vi "Script RPC Client VI.vi"(6 "rpc method parameters":T1, 7 "owning library":refnum<vi>, 8 "error in (no error)":errorcluster, 9 "rpc service name":string, 10 "owning folder":refnum<vi>, 11 "template project item":refnum<vi>) -> (0 "error out":errorcluster)   [LabVIEW 2019, in "gRPC Template Creation Utility.lvlib"]
uses:
  gRPC Template Creation Utility.lvlib
  TypeDefs/RPC Method Parameters.ctl
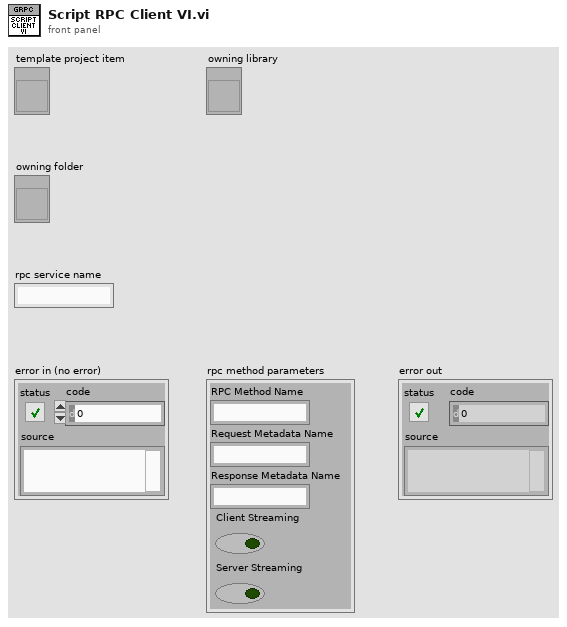
[diagram p1: front panel]
types:
  T1 = typedef "gRPC Template Creation Utility.lvlib/RPC Method Parameters.ctl" = cluster{"RPC Method Name":string, "Request Metadata Name":string, "Response Metadata Name":string, "Client Streaming":bool, "Server Streaming":bool}
  T2 = enum32{"invalid VI type", "Standard VI", "Control VI", "Global VI", "Polymorphic VI", "Configuration VI", "SubSystem", "Facade VI", "Method VI"}
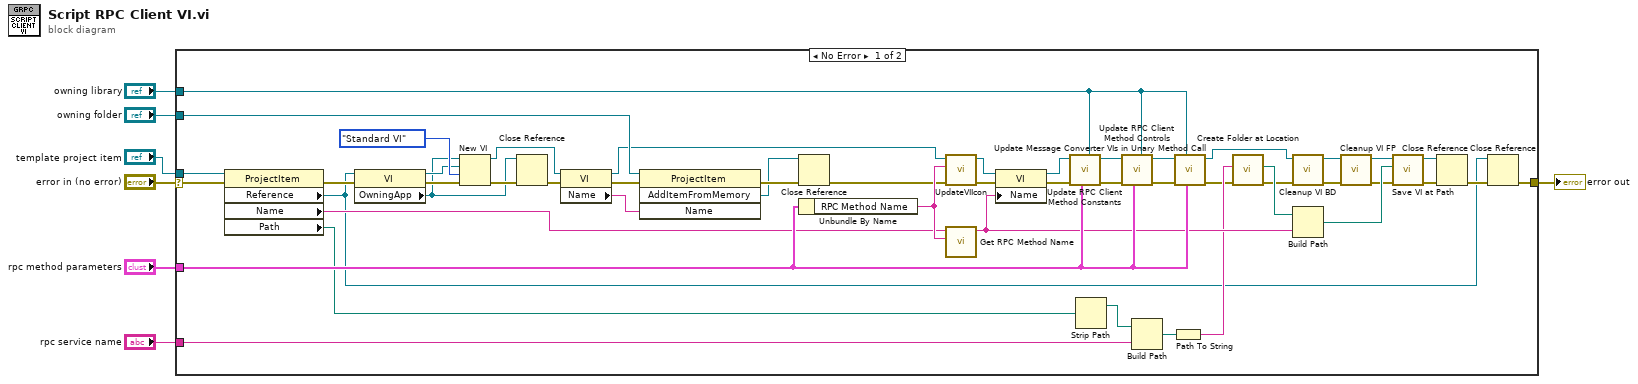
[diagram p0: block diagram]
diagram:
  n1 = case shown="No Error" "error in (no error)" {
    selector: "error in (no error)" -> [w29 w57]
    tunnel: "rpc method parameters" -> [w56 _]
    tunnel: "owning library" -> [w55 _]
    tunnel: [w12 w57] -> w5
    tunnel: "rpc service name" -> [w43 _]
    tunnel: "owning folder" -> [w41 _]
    tunnel: "template project item" -> [w32 _]
    frame No Error {
      n2 = property class="ProjectItem"(reference=w32, error in=w29) -> (error out=w16:errorcluster, "Reference"=w11:refnum<vi>, "Name"=w31:string, "Path"=w30:path)  [unwired: 1 out]
      n3 = property class="VI"(reference=w11, error in=w16) -> (reference out=w14:refnum<vi>, error out=w15:errorcluster, "OwningApp"=w8:refnum<vi>)
      n4 = New VI(8:w15, 9:T2."Standard VI" ("vi type (standard vi)"), 10:w14, 11:w8) -> (0:w10:errorcluster, 3:w28:refnum<vi>)  [unwired: 3 out]
      n5 = Close Reference(reference=w8, error in (no error)=w10) -> (error out=w9:errorcluster)
      n6 = property class="VI"(reference=w28, error in=w9) -> (reference out=w27:refnum<vi>, error out=w35:errorcluster, "Name"=w33:string)
      n7 = invoke class="ProjectItem" method="AddItemFromMemory"(reference=w41, error in=w35, "Name"=w33) -> (error out=w40:errorcluster, "AddItemFromMemory"=w39:refnum<vi>)  [unwired: 1 in, 2 out]
      n8 = Close Reference(reference=w39, error in (no error)=w40) -> (error out=w24:errorcluster)
      n9 = Unbundle By Name(w56) -> ("RPC Method Name"=w52:string)
      n10 = call "UpdateVIIcon.vi"("error in (no error)"=w24, "Method Name"=w52, "VI in"=w27) -> ("error out"=w25:errorcluster, "VI out"=w26:refnum<vi>)  [unwired: 7 in]
      n11 = call "Get RPC Method Name.vi"("RPC Method Name"=w52, "Template VI Name"=w31) -> ("RPC VI Name"=w51:string)  [unwired: 8 in, 1 out]
      n12 = property class="VI"(reference=w26, error in=w25, "Name"=w51) -> (reference out=w49:refnum<vi>, error out=w47:errorcluster)
      n13 = call "Update RPC Client Method Constants.vi"("Library"=w55, "RPC Method Parameters"=w56, "error in (no error)"=w47, "VI in"=w49) -> ("error out"=w48:errorcluster, "VI out"=w50:refnum<vi>)  [unwired: 6 in]
      n14 = Strip Path(path=w30) -> (stripped path=w42:path)  [unwired: 1 out]
      n15 = call "Update RPC Client Method Controls.vi"("Library"=w55, "RPC Method Parameters"=w56, "error in (no error)"=w48, "VI in"=w50) -> ("error out"=w54:errorcluster, "VI out"=w53:refnum<vi>)  [unwired: 6 in]
      n16 = Build Path(base path=w42, name or relative path=w43) -> (appended path=w44:path)
      n17 = Path To String(path=w44) -> (string=w45:string)
      n18 = call "Update Message Converter VIs in Unary Method Call.vi"("RPC Method Parameters"=w56, "Library"=w55, "error in (no error)"=w54, "VI in"=w53) -> ("error out"=w23:errorcluster, "VI out"=w20:refnum<vi>)  [unwired: 6 in]
      n19 = call "Create Folder at Location.vi"("Error In"=w23, "Path"=w45) -> ("Error Out"=w18:errorcluster, "Full path out"=w46:path)  [unwired: 7 in, 1 out]
      n20 = call "Cleanup VI BD.vi"("error in (no error)"=w18, "VI in"=w20) -> ("error out"=w22:errorcluster, "VI out"=w21:refnum<vi>)  [unwired: 8 in]
      n21 = Build Path(base path=w46, name or relative path=w51) -> (appended path=w36:path)
      n22 = call "Cleanup VI FP.vi"("error in"=w22, "vi in"=w21) -> ("error out"=w17:errorcluster, "vi out"=w19:refnum<vi>)  [unwired: 8 in]
      n23 = call "Save VI at Path.vi"("error in (no error)"=w17, "Path"=w36, "VI in"=w19) -> ("error out"=w37:errorcluster, "VI out"=w38:refnum<vi>)  [unwired: 6 in, 1 out]
      n24 = Close Reference(reference=w38, error in (no error)=w37) -> (error out=w13:errorcluster)
      n25 = Close Reference(reference=w11, error in (no error)=w13) -> (error out=w12:errorcluster)
    }
    frame Error {
    }
  }
  "error out" <- w5
